vi "query LTE Bandwidth.vi"(8 "error in (no error)":errorcluster, 9 "LTE Channel Type":T2, 11 "Anritsu Call Box_Implement in":refnum<class "Anritsu Call Box_Implement.lvclass">) -> (0 "error out":errorcluster, 2 "BandWidth":T1, 3 "Anritsu Call Box_Implement out":refnum<class "Anritsu Call Box_Implement.lvclass">)   [LabVIEW 2023, in "ANRITSU Call Box.lvlib" / "Anritsu Call Box_Implement.lvclass"]
uses:
  Anritsu Call Box_Implement.lvclass
  Anritsu Call Box_Implement.lvclass/Anritsu Call Box_Implement.ctl
  LTE/LTE.lvclass
  Type Definition/LTE Channel Type.ctl
  ANRITSU Call Box.lvlib
  Type Definition/LTE Supported BandWidth.ctl
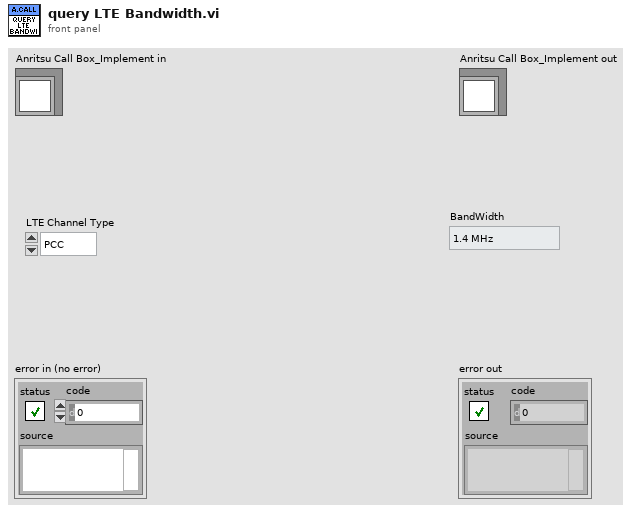
[diagram p1: front panel]
types:
  T1 = typedef "ANRITSU Call Box.lvlib/LTE Supported BandWidth.ctl" = enum16{"1.4 MHz", "3 MHz", "5 MHz", "10 MHz", "15 MHz", "20 MHz"}
  T2 = typedef "ANRITSU Call Box.lvlib/LTE Channel Type.ctl" = enum16{"PCC", "SCC1", "SCC2", "SCC3"}
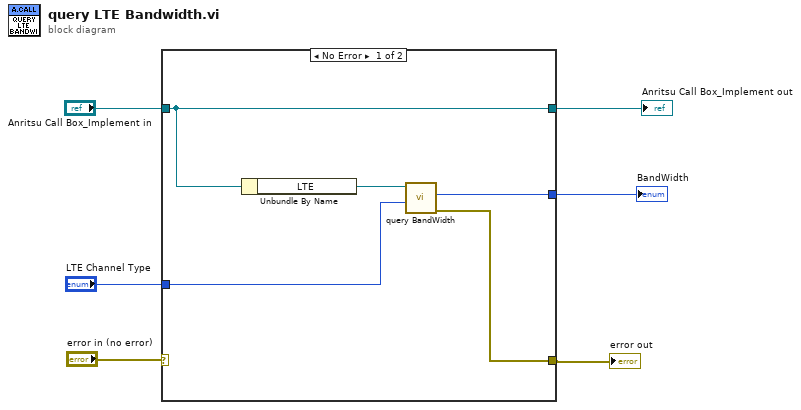
[diagram p0: block diagram]
diagram:
  n1 = case shown="No Error" "error in (no error)" {
    selector: "error in (no error)" -> [_ w12]
    tunnel: "Anritsu Call Box_Implement in" -> [w11 w13]
    tunnel: [w11 w13] -> w5
    tunnel: [w8 w12] -> w2
    tunnel: "LTE Channel Type" -> [w9 _]
    tunnel: [w7 _] -> w1
    frame No Error {
      n2 = Unbundle By Name(w11) -> ("LTE"=w10:refnum<class "LTE.lvclass">)
      n3 = call "query BandWidth.vi"("LTE Channel Type"=w9, "LTE in"=w10) -> ("error out"=w8:errorcluster, "BandWidth"=w7:T1)  [unwired: 7 in, 1 out]
    }
    frame Error {
    }
  }
  "error out" <- w2
  "Anritsu Call Box_Implement out" <- w5
  "BandWidth" <- w1
